vi "Save into new sequence.vi"(5 "number of images to save":u32, 7 "First image to save (start with 0)":u32, 9 "Header2 file data":T1, 10 "Header file data":T2 {"Pixel depth" items=["8 bits", "16 bits", "Float", "Complex", "RGB", "HSL"]; "time of 1st frame, \nsec since 1/1/04" format="%.2f"}, 11 "Acquisition refnum array":refnum<file>[](array[refnum])) -> ()   [LabVIEW 2015]
uses:
  Header file data.ctl
  Seq file v 1/Offset table.ctl
  Seq file v 1/Offset.ctl
  Seq file v 1/file number.ctl
  Header2 file data.ctl
  GLIMPSE Globals.vi
panel:
  out "Input sequence  frame number":i32(slide) scale=1.0..13.0
  in  "error in":errorcluster
  out "Save into new directory:":path=path "d:/1.glimpse"
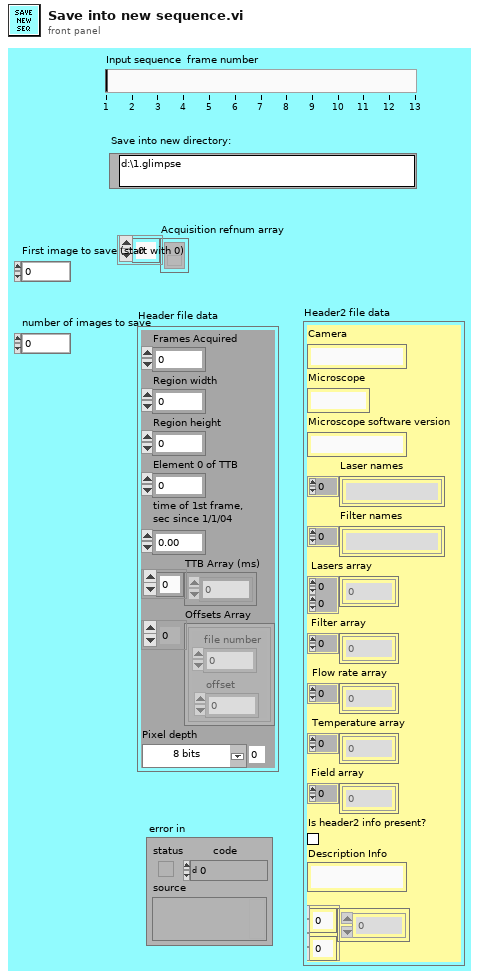
[diagram p1: front panel]
types:
  T1 = typedef "Header2 file data.ctl" = cluster{"Camera":string, "Microscope":string, "Microscope software version":string, "Laser names":string[], "Filter names":string[], "Lasers array":u16[][], "Filter array":u16[], "Flow rate array":dbl[], "Temperature array":dbl[], "Field array":u16[], "Is header2 info present?":bool, "Description Info":string, "Stage xyz array":dbl[][]}
  T2 = typedef "Header file data.ctl" = cluster{"Frames Acquired":u32, "Region width":i32, "Region height":i32, "Element 0 of TTB":u32, "time of 1st frame, \nsec since 1/1/04":dbl, "TTB Array (ms)":u32[], "Offsets Array":T3, "Pixel depth":u32}
  T3 = typedef "Offset table.ctl" = cluster{"offset":T4, "file number":T5}[]
  T4 = typedef "Offset.ctl" = i32
  T5 = typedef "file number.ctl" = u8
  T6 = typedef "IMAQ Image.ctl" = refnum<image>
  T7 = typedef "Sequence files handle.ctt" = cluster{"Sequence files directory path":path, "Sequence files refnum array":refnum<file>[]}
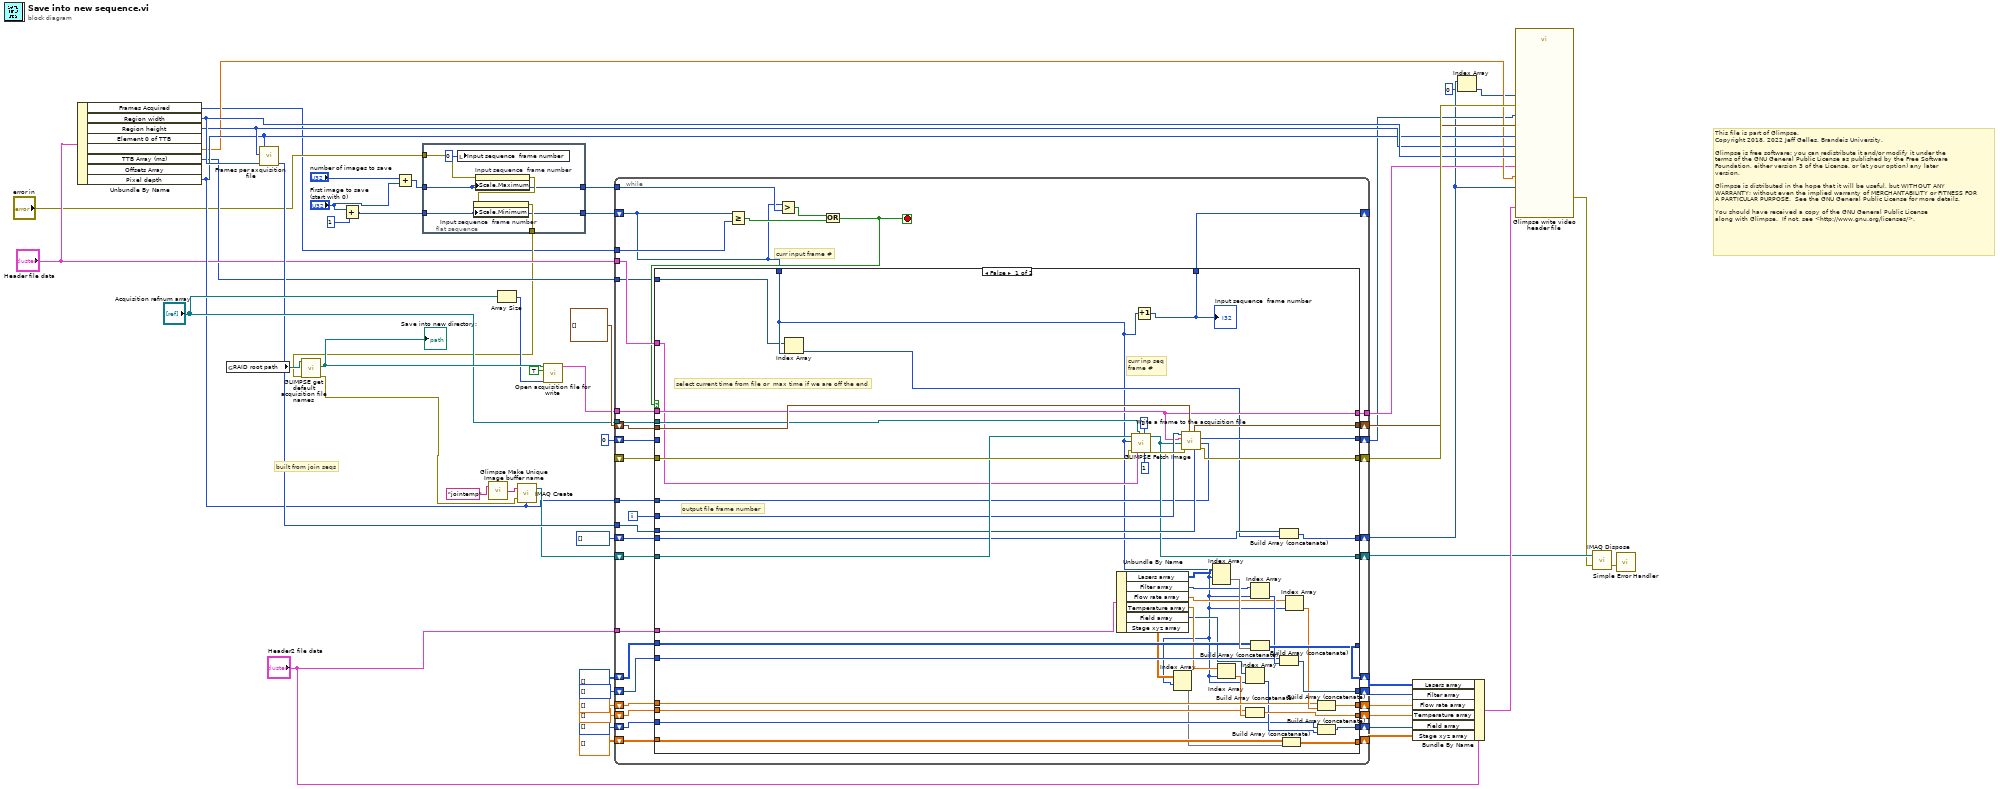
[diagram p0: block diagram]
diagram:
  # "built from join seqs"
  # "This file is part of Glimpse. \nCopyright 2018, 2022 Jeff Gelles, Brandeis University.    \n\nGlimpse is free software: you can redistribute it and/or modify it under the \nterms of the GNU General Public License as published by the Free Software \nFoundation, either version 3 of the License, or (at your option) any later \nversion.\n\nGlimpse is distributed in the hope that it will be useful, but WITHOUT ANY \nWARRANTY; without even the implied warranty of MERCHANTABILITY or FITNESS FOR \nA PARTICULAR PURPOSE.  See the GNU General Public License for more details.\n\nYou should have received a copy of the GNU General Public License\nalong with Glimpse.  If not, see <http://www.gnu.org/licenses/>."
  n1 = Unbundle By Name("Header file data") -> ("Frames Acquired"=w6:u32, "Region width"=w21:i32, "Region height"=w20:i32, "time of 1st frame, \nsec since 1/1/04"=w12:dbl, "TTB Array (ms)"=w17:u32[], "Pixel depth"=w19:u32)  [unwired: 2 out]
  n2 = global read "GLIMPSE Globals.vi" "RAID root path"() -> (w54:path)
  n3 = call "Frames per axquisition file.vi"("Output frame width"=w21, "Output frame height"=w20, "Pixel depth"=w19) -> ("Frames per acquisition file"=w38:i32)  [unwired: 3 in, 1 out]
  n4 = call "GLIMPSE get default acquisition file names.vi"("error in"=w13, "RAID root path"=w54) -> ("error out"=w35:errorcluster, "next directory path"=w53:path)  [unwired: 6 out]
  "Save into new directory:" <- w53
  n5 = Add(x="First image to save (start with 0)", y=u32 1) -> (x+y=w4:u32)
  n6 = Add(x="number of images to save", y="First image to save (start with 0)") -> (x+y=w3:u32)
  n7 = flat-sequence {
    tunnel: [w56] -> w16
    tunnel: [w55] -> w15
    tunnel: "error in" -> [w59]
    tunnel: [w57] -> w13
    tunnel: w4 -> [w56]
    tunnel: w3 -> [w55]
    frame #0 {
      n8 = local write "Input sequence  frame number"(0 ("Input sequence  frame number")) -> ()
      n9 = property on="Input sequence  frame number" class="Slide (strict)"(error in=w59, "Scale.Maximum"=w55) -> (error out=w58:errorcluster)  [unwired: 1 in, 1 out]
      n10 = property on="Input sequence  frame number" class="Slide (strict)"(error in=w58, "Scale.Minimum"=w56) -> (error out=w57:errorcluster)  [unwired: 1 in, 1 out]
    }
  }
  n11 = call "Glimpse Make Unique Image buffer name.vi"("Buffer  base name"="jointemp" ("Image Name")) -> ("Image Name"=w37:string)  [unwired: 1 out]
  n12 = Array Size(array="Acquisition refnum array") -> (size(s)=w51:i32)
  n13 = call "IMAQ Create"("Image Name"=w37, "Image Type"=w19, "error in (no error)"=w35) -> ("New Image"=w34:T6)  [unwired: 1 in, 2 out]
  n14 = call "Open acquisition file for write.vi"("Number of acquisition files"=w51, "Use new?"=TRUE, "New directory to create"=w53) -> ("Sequence files handle"=w41:T7)  [unwired: 1 in, 6 out]
  n15 = while {
    tunnel: "Header file data" -> [w98]
    shift-right: [w88] -> _
    shift-left: w16 -> [w61]
    tunnel: "Acquisition refnum array" -> [w97]
    shift-right: [w95] -> w33
    shift-left: _ -> [w96]
    shift-right: [w87] -> w32
    shift-left: w34 -> [w94]
    tunnel: w41 -> [w93]
    shift-right: [w91] -> w22
    shift-left: cluster{"offset":i32, "file number":u8}[] [] ("Offset table out") -> [w90]
    tunnel: w38 -> [w89]
    shift-right: [w86] -> w9
    shift-left: u32[] [] -> [w85]
    shift-right: [w84] -> w10
    shift-left: u32 0 ("Last frame number written out") -> [w83]
    tunnel: [w82] -> w11
    shift-right: [w81] -> w28
    shift-left: u16[][] [] -> [w80]
    shift-right: [w79] -> w27
    shift-left: u16[] [] -> [w78]
    shift-right: [w77] -> w26
    shift-left: dbl[] [] -> [w76]
    shift-right: [w75] -> w25
    shift-left: dbl[] [] -> [w74]
    shift-right: [w73] -> w24
    shift-left: u16[] [] -> [w72]
    shift-right: [w70] -> w23
    shift-left: dbl[][] [] -> [w71]
    tunnel: "Header2 file data" -> [w69]
    tunnel: w19 -> [w68]
    tunnel: w6 -> [w64]
    tunnel: w17 -> [w63]
    tunnel: w15 -> [w62]
    i -> [w92]
    stop <- w65 stop-if-true
    # "curr input frame #"
    n16 = Greater Or Equal?(x=w61, y=w64) -> (x >= y?=w67:bool)
    n17 = Greater?(x=w61, y=w62) -> (0:w66:bool)
    n18 = Or(x=w66, y=w67) -> (x .or. y?=w65:bool)
    n19 = case shown="False" w65 {
      tunnel: w98 -> [w105 _]
      tunnel: w61 -> [w101 w152]
      tunnel: w97 -> [w106 _]
      tunnel: w96 -> [w145 w156]
      tunnel: [w140 w156] -> w95
      tunnel: w94 -> [w142 w154]
      tunnel: w93 -> [w132 w153]
      tunnel: w92 -> [w139 _]
      tunnel: [w138 w158] -> w91
      tunnel: w90 -> [w137 w158]
      tunnel: w89 -> [w136 _]
      tunnel: [w100 w152] -> w88
      tunnel: [w135 w154] -> w87
      tunnel: [w134 w155] -> w86
      tunnel: w85 -> [w133 w155]
      tunnel: [w131 w157] -> w84
      tunnel: w83 -> [_ w157]
      tunnel: [w132 w153] -> w82
      tunnel: [w128 w151] -> w81
      tunnel: w80 -> [w127 w151]
      tunnel: [w124 w150] -> w79
      tunnel: w78 -> [w123 w150]
      tunnel: [w114 w149] -> w77
      tunnel: w76 -> [w120 w149]
      tunnel: [w118 w148] -> w75
      tunnel: w74 -> [w116 w148]
      tunnel: [w113 w147] -> w73
      tunnel: w72 -> [w111 w147]
      tunnel: w71 -> [w110 w146]
      tunnel: [w107 w146] -> w70
      tunnel: w69 -> [w104 _]
      tunnel: w68 -> [w103 _]
      tunnel: w63 -> [w99 _]
      frame False {
        # "select current time from file or  max time if we are off the end"
        # "output file frame number"
        # "curr inp seq\nframe #"
        n20 = Index Array(array=w99, index=w101) -> (element=w102:u32)
        n21 = Unbundle By Name(w104) -> ("Lasers array"=w130:u16[][], "Filter array"=w126:u16[], "Flow rate array"=w122:dbl[], "Temperature array"=w119:dbl[], "Field array"=w115:u16[], "Stage xyz array"=w109:dbl[][])
        n22 = call "GLIMPSE Fetch Image.vi"("Display FOV number"=i16 1, "Total FOVs"=i16 1, "Header file data"=w105, "Acqisition files refnums"=w106, "error in"=w145, "Logical Frame Number\n(starting with zero)"=w101, "Image In"=w142) -> ("error out"=w141:errorcluster, "Image Out"=w135:T6)  [unwired: 2 in, 1 out]
        n23 = Increment(x=w101) -> (x+1=w100:u32)
        "Input sequence  frame number" <- w100
        n24 = Index Array(array=w109, index (row)=w101) -> (element=w108:dbl[])  [unwired: 1 in]
        n25 = call "Write a frame to the acquisition file.vi"("Pixel depth"=w103, "Frames per acquisition file"=w136, "Offset table in"=w137, "error in"=w141, "Image In"=w135, "Sequence files handle"=w132, "Last frame number written in"=w139) -> ("error out"=w140:errorcluster, "Last frame number written out"=w131:u32, "Offset table out"=w138:T3)  [unwired: 2 out]
        n26 = Index Array(array=w130, index (row)=w101) -> (element=w129:u16[])  [unwired: 1 in]
        n27 = Index Array(array=w119, index=w101) -> (element=w117:dbl)
        n28 = Index Array(array=w115, index=w101) -> (element=w112:u16)
        n29 = Build Array (concatenate)(w116, w117) -> (w118:dbl[])
        n30 = Index Array(array=w126, index=w101) -> (element=w125:u16)
        n31 = Build Array (concatenate)(w127, w129) -> (w128:u16[][])
        n32 = Build Array (concatenate)(w133, w102) -> (w134:u32[])
        n33 = Build Array (concatenate)(w123, w125) -> (w124:u16[])
        n34 = Build Array (concatenate)(w110, w108) -> (w107:dbl[][])
        n35 = Index Array(array=w122, index=w101) -> (element=w121:dbl)
        n36 = Build Array (concatenate)(w120, w121) -> (w114:dbl[])
        n37 = Build Array (concatenate)(w111, w112) -> (w113:u16[])
      }
      frame True {
      }
    }
  }
  n38 = Bundle By Name(cluster="Header2 file data", "Lasers array"=w28, "Filter array"=w27, "Flow rate array"=w26, "Temperature array"=w25, "Field array"=w24, "Stage xyz array"=w23) -> (w40:T1)
  n39 = Index Array(array=w9, index=0) -> (element=w7:u32)
  n40 = call "Glimpse write video header file.vi"("Number of frames"=w10, "Sequence files handle"=w11, "Pixel depth\n(0=8 bit; 1= 16 bit)"=w19, "error in"=w33, "TTB Array"=w9, "Offsets Array"=w22, "Header2 file data"=w40, "Region width"=w21, "Region height"=w20, "Element 0 of TTB"=w7, "time of 1st frame, \nsec since 1/1/04"=w12) -> ("error out"=w31:errorcluster)  [unwired: 8 in]
  n41 = call "IMAQ Dispose"("Image"=w32, "error in (no error)"=w31) -> ("error out"=w30:errorcluster)  [unwired: 1 in, 3 out]
  n42 = call <vilib>:"Simple Error Handler.vi"("error in (no error)"=w30) -> ()  [unwired: 4 in, 5 out]
